vi "Restore Data.vi"(8 "error in (no error)":errorcluster caption="错误输入（无错误）", 11 "Data Viewer 输入":refnum<class "Data Viewer.lvclass">) -> (0 "error out":errorcluster caption="错误输出", 3 "Data Viewer 输出":refnum<class "Data Viewer.lvclass">)   [LabVIEW 2020, in "Data Viewer.lvlib" / "Data Viewer.lvclass"]
uses:
  Data Viewer.lvclass
  Data Viewer.lvclass/Data Viewer.ctl
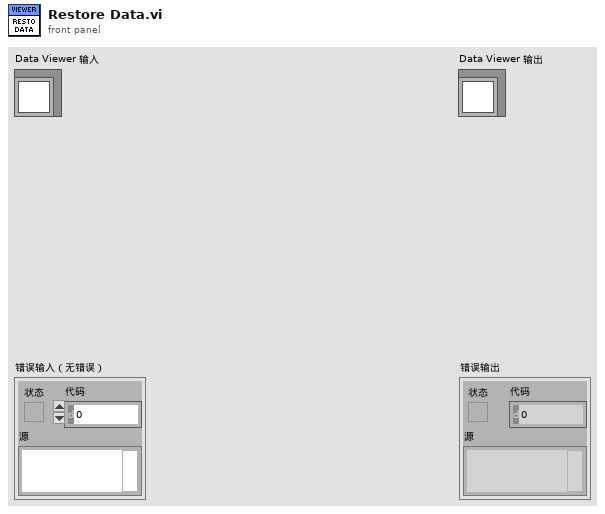
[diagram p1: front panel]
types:
  T1 = typedef "Data Viewer.lvlib/Data Serie--cluster.ctl" = cluster{"Name":string, "Unit":string, "Sample Rate[Hz]":dbl, "Delta t[S]":dbl, "t0":timestamp, "Length":i32, "Time":timestamp[], "Value":dbl[]}
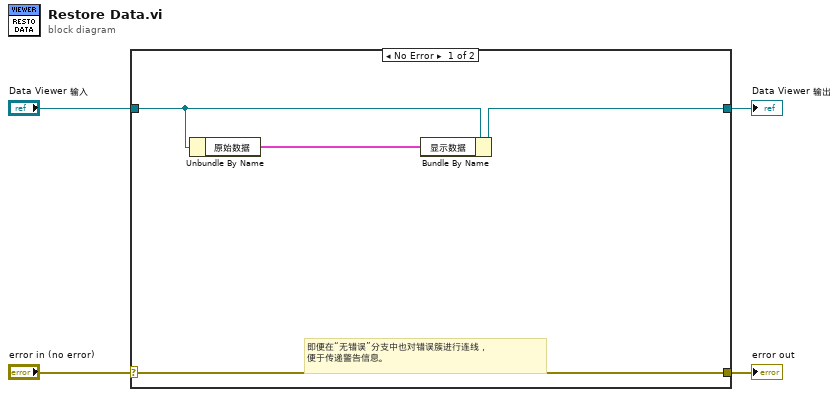
[diagram p0: block diagram]
diagram:
  n1 = case shown="No Error" "error in (no error)" {
    selector: "error in (no error)" -> [w8 w10]
    tunnel: [w8 w10] -> w3
    tunnel: [w6 w9] -> w1
    tunnel: "Data Viewer 输入" -> [w7 w9]
    frame No Error {
      # "即便在“无错误”分支中也对错误簇进行连线，\n便于传递警告信息。"
      n2 = Unbundle By Name(w7) -> ("原始数据"=w5:T1[])
      n3 = Bundle By Name(cluster=w7, "显示数据"=w5) -> (w6:refnum<class "Data Viewer.lvclass">)
    }
    frame Error {
    }
  }
  "error out" <- w3
  "Data Viewer 输出" <- w1
